vi "Test_Advance_Step_Caraya.vi"(8 "error in":errorcluster) -> (0 "error out":errorcluster)   [LabVIEW 2026]
doc: "Caraya tests of the configurable step phase logic."
uses:
  <vilib>/addons/_JKI Toolkits/Caraya/classes/Test/Test.lvclass
  <vilib>/addons/_JKI Toolkits/Caraya/classes/Assert/Assert.lvclass
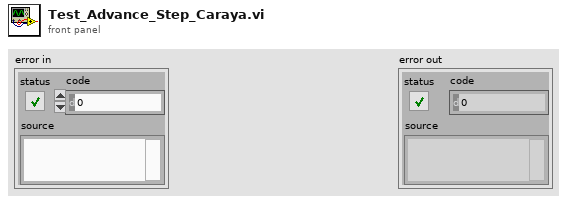
[diagram p1: front panel]
types:
  T1 = cluster{"phase":i32, "phase_start_ms":dbl, "retries":i32}
  T2 = cluster{"step_no":i32, "step_name":string, "interlock_status":string, "pre_delay_ms":dbl, "post_delay_ms":dbl, "timeout_ms":dbl, "popup":cluster{"enabled":bool, "message":string, "type":string, "timeout_ms":dbl}, "retest":cluster{"enabled":bool, "popup":bool, "popup_message":string, "condition":string, "goto_step_no":i32}, "log":cluster{"peak":bool, "average":bool, "event":bool}, "actions":cluster{"do":cluster{"name":string, "on":bool, "mode":string}[], "ao":cluster{"name":string, "value":dbl, "mode":string}[], "misc_write":cluster{"name":string, "on":bool}[], "call":string[]}, "checks":cluster{"di_high":cluster{"and":string[], "or":string[]}, "di_low":cluster{"and":string[], "or":string[]}, "misc_high":cluster{"and":string[], "or":string[]}, "misc_low":cluster{"and":string[], "or":string[]}, "t0_high":cluster{"and":cluster{"name":string, "min":dbl, "max":dbl}[], "or":cluster{"name":string, "min":dbl, "max":dbl}[]}, "t0_low":cluster{"and":cluster{"name":string, "min":dbl, "max":dbl}[], "or":cluster{"name":string, "min":dbl, "max":dbl}[]}, "misc_compare":cluster{"name":string, "compare_with":string, "comparison":string, "tolerance":dbl}[]}}
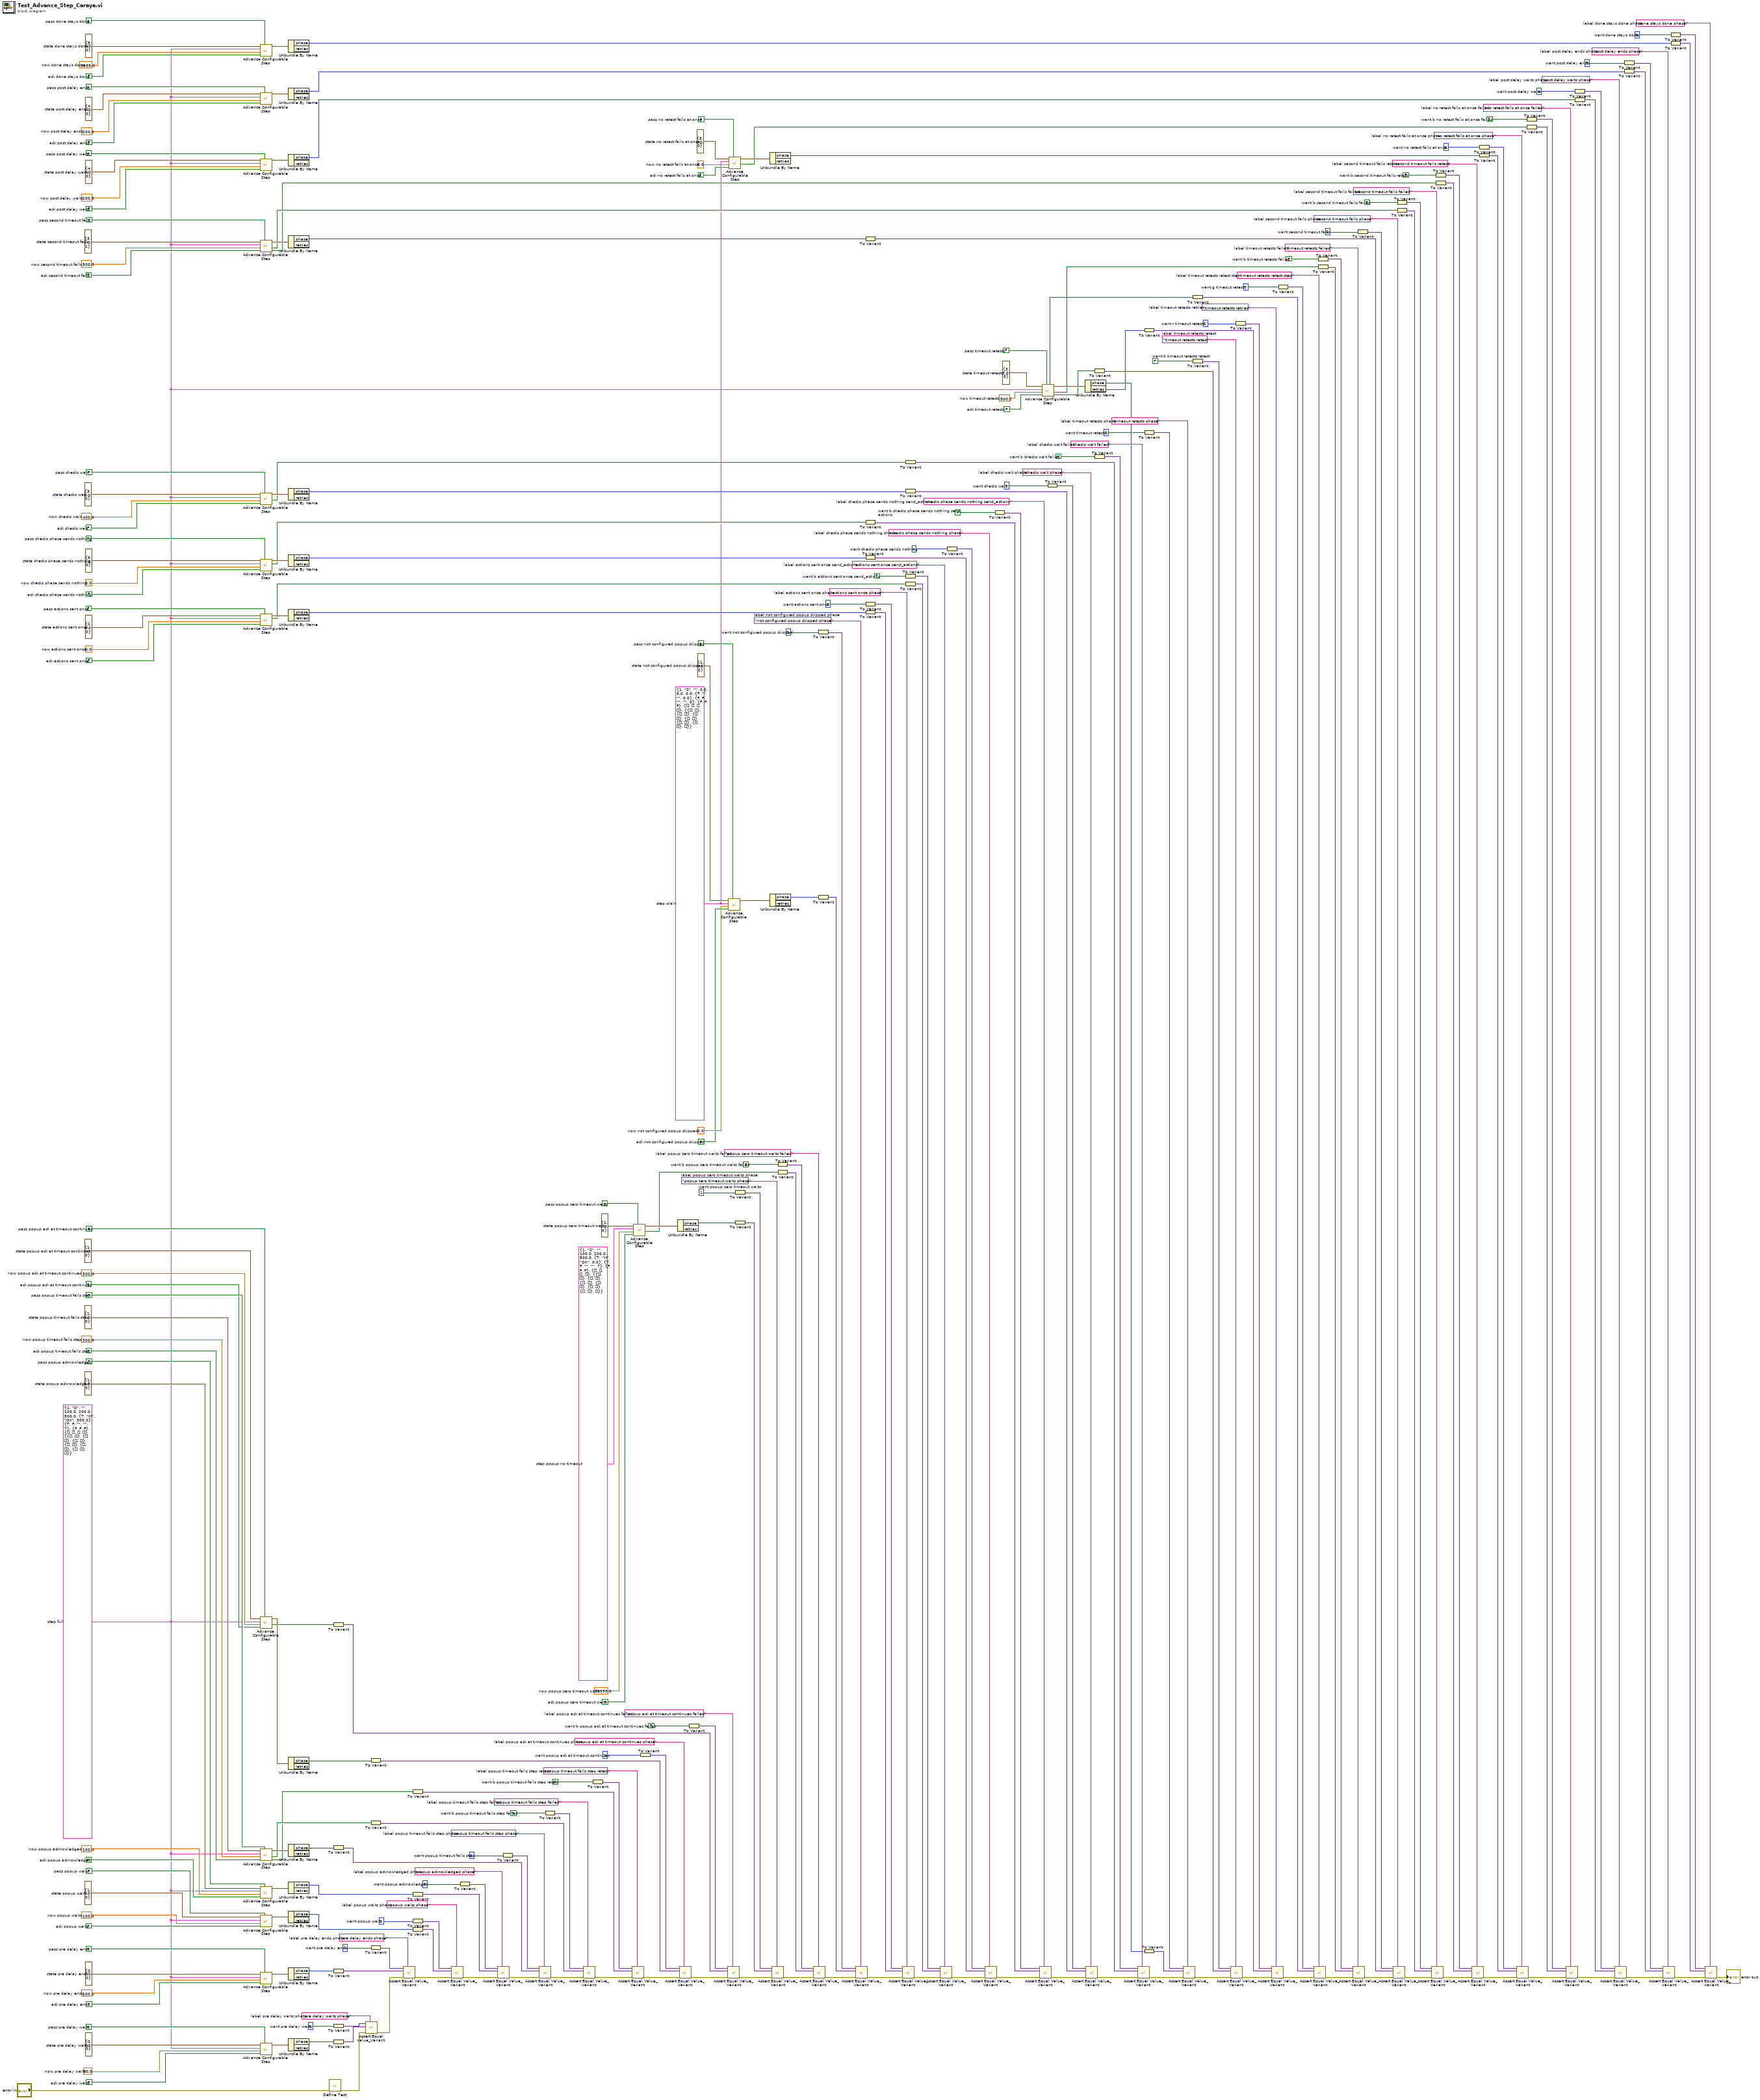
[diagram p0: block diagram]
diagram:
  w5 = "done stays done phase"  # label done stays done phase
  w6 = 5  # want done stays done
  w9 = FALSE  # pass done stays done
  w10 = FALSE  # ack done stays done
  w11 = 9999.0  # now done stays done
  w13 = T1 {"phase"=5, "phase_start_ms"=0.0, "retries"=0}  # state done stays done
  w17 = "post delay ends phase"  # label post delay ends phase
  w18 = 5  # want post delay ends
  w21 = FALSE  # pass post delay ends
  w22 = FALSE  # ack post delay ends
  w23 = 200.0  # now post delay ends
  w24 = T1 {"phase"=4, "phase_start_ms"=0.0, "retries"=0}  # state post delay ends
  w28 = "post delay waits phase"  # label post delay waits phase
  w29 = 4  # want post delay waits
  w32 = FALSE  # pass post delay waits
  w33 = FALSE  # ack post delay waits
  w34 = 100.0  # now post delay waits
  w35 = T1 {"phase"=4, "phase_start_ms"=0.0, "retries"=0}  # state post delay waits
  w39 = "no retest fails at once failed"  # label no retest fails at once failed
  w40 = TRUE  # want b no retest fails at once failed
  w45 = "no retest fails at once phase"  # label no retest fails at once phase
  w46 = 6  # want no retest fails at once
  w49 = FALSE  # pass no retest fails at once
  w50 = FALSE  # ack no retest fails at once
  w51 = 0.0  # now no retest fails at once
  w53 = T1 {"phase"=3, "phase_start_ms"=0.0, "retries"=0}  # state no retest fails at once
  w57 = "second timeout fails retest"  # label second timeout fails retest
  w58 = FALSE  # want b second timeout fails retest
  w63 = "second timeout fails failed"  # label second timeout fails failed
  w64 = TRUE  # want b second timeout fails failed
  w69 = "second timeout fails phase"  # label second timeout fails phase
  w70 = 6  # want second timeout fails
  w73 = FALSE  # pass second timeout fails
  w74 = FALSE  # ack second timeout fails
  w75 = 500.0  # now second timeout fails
  w76 = T1 {"phase"=3, "phase_start_ms"=0.0, "retries"=1}  # state second timeout fails
  w80 = "timeout retests failed"  # label timeout retests failed
  w81 = FALSE  # want b timeout retests failed
  w86 = "timeout retests retest step"  # label timeout retests retest step
  w87 = 7  # want g timeout retests
  w92 = "timeout retests retries"  # label timeout retests retries
  w93 = 1  # want r timeout retests
  w98 = "timeout retests retest"  # label timeout retests retest
  w99 = TRUE  # want b timeout retests retest
  w104 = "timeout retests phase"  # label timeout retests phase
  w105 = 0  # want timeout retests
  w108 = FALSE  # pass timeout retests
  w109 = FALSE  # ack timeout retests
  w110 = 500.0  # now timeout retests
  w111 = T1 {"phase"=3, "phase_start_ms"=0.0, "retries"=0}  # state timeout retests
  w115 = "checks wait failed"  # label checks wait failed
  w116 = FALSE  # want b checks wait failed
  w121 = "checks wait phase"  # label checks wait phase
  w122 = 3  # want checks wait
  w125 = FALSE  # pass checks wait
  w126 = FALSE  # ack checks wait
  w127 = 400.0  # now checks wait
  w128 = T1 {"phase"=3, "phase_start_ms"=0.0, "retries"=0}  # state checks wait
  w132 = "checks phase sends nothing send_actions"  # label checks phase sends nothing send_actions
  w133 = FALSE  # want b checks phase sends nothing send_actions
  w138 = "checks phase sends nothing phase"  # label checks phase sends nothing phase
  w139 = 4  # want checks phase sends nothing
  w142 = TRUE  # pass checks phase sends nothing
  w143 = FALSE  # ack checks phase sends nothing
  w144 = 0.0  # now checks phase sends nothing
  w145 = T1 {"phase"=3, "phase_start_ms"=0.0, "retries"=0}  # state checks phase sends nothing
  w149 = "actions sent once send_actions"  # label actions sent once send_actions
  w150 = TRUE  # want b actions sent once send_actions
  w155 = "actions sent once phase"  # label actions sent once phase
  w156 = 3  # want actions sent once
  w159 = FALSE  # pass actions sent once
  w160 = FALSE  # ack actions sent once
  w161 = 0.0  # now actions sent once
  w162 = T1 {"phase"=2, "phase_start_ms"=0.0, "retries"=0}  # state actions sent once
  w166 = "not configured popup skipped phase"  # label not configured popup skipped phase
  w167 = 2  # want not configured popup skipped
  w170 = FALSE  # pass not configured popup skipped
  w171 = FALSE  # ack not configured popup skipped
  w172 = 0.0  # now not configured popup skipped
  w173 = T1 {"phase"=1, "phase_start_ms"=0.0, "retries"=0}  # state not configured popup skipped
  w177 = "popup zero timeout waits failed"  # label popup zero timeout waits failed
  w178 = FALSE  # want b popup zero timeout waits failed
  w183 = "popup zero timeout waits phase"  # label popup zero timeout waits phase
  w184 = 1  # want popup zero timeout waits
  w187 = FALSE  # pass popup zero timeout waits
  w188 = FALSE  # ack popup zero timeout waits
  w189 = 99999.0  # now popup zero timeout waits
  w191 = T1 {"phase"=1, "phase_start_ms"=0.0, "retries"=0}  # state popup zero timeout waits
  w190 = T2 {"step_no"=1, "step_name"="S", "interlock_status"="", "pre_delay_ms"=100.0, "post_delay_ms"=200.0, "timeout_ms"=500.0, "popup"={"enabled"=TRUE, "message"="M", "type"="OK", "timeout_ms"=0.0}, "retest"={"enabled"=TRUE, "popup"=FALSE, "popup_message"="", "condition"="", "goto_step_no"=7}, "log"={"peak"=FALSE, "average"=FALSE, "event"=FALSE}, "actions"={"do"=[], "ao"=[], "misc_write"=[], "call"=[]}, "checks"={"di_high"={"and"=[], "or"=[]}, "di_low"={"and"=[], "or"=[]}, "misc_high"={"and"=[], "or"=[]}, "misc_low"={"and"=[], "or"=[]}, "t0_high"={"and"=[], "or"=[]}, "t0_low"={"and"=[], "or"=[]}, "misc_compare"=[]}}  # step popup no timeout
  w195 = "popup ack at timeout continues failed"  # label popup ack at timeout continues failed
  w196 = FALSE  # want b popup ack at timeout continues failed
  w201 = "popup ack at timeout continues phase"  # label popup ack at timeout continues phase
  w202 = 2  # want popup ack at timeout continues
  w205 = FALSE  # pass popup ack at timeout continues
  w206 = TRUE  # ack popup ack at timeout continues
  w207 = 300.0  # now popup ack at timeout continues
  w208 = T1 {"phase"=1, "phase_start_ms"=0.0, "retries"=0}  # state popup ack at timeout continues
  w212 = "popup timeout fails step retest"  # label popup timeout fails step retest
  w213 = FALSE  # want b popup timeout fails step retest
  w218 = "popup timeout fails step failed"  # label popup timeout fails step failed
  w219 = TRUE  # want b popup timeout fails step failed
  w224 = "popup timeout fails step phase"  # label popup timeout fails step phase
  w225 = 6  # want popup timeout fails step
  w228 = FALSE  # pass popup timeout fails step
  w229 = FALSE  # ack popup timeout fails step
  w230 = 300.0  # now popup timeout fails step
  w231 = T1 {"phase"=1, "phase_start_ms"=0.0, "retries"=0}  # state popup timeout fails step
  w235 = "popup acknowledged phase"  # label popup acknowledged phase
  w236 = 2  # want popup acknowledged
  w239 = FALSE  # pass popup acknowledged
  w240 = TRUE  # ack popup acknowledged
  w241 = 100.0  # now popup acknowledged
  w242 = T1 {"phase"=1, "phase_start_ms"=0.0, "retries"=0}  # state popup acknowledged
  w246 = "popup waits phase"  # label popup waits phase
  w247 = 1  # want popup waits
  w250 = FALSE  # pass popup waits
  w251 = FALSE  # ack popup waits
  w252 = 100.0  # now popup waits
  w253 = T1 {"phase"=1, "phase_start_ms"=0.0, "retries"=0}  # state popup waits
  w257 = "pre delay ends phase"  # label pre delay ends phase
  w258 = 1  # want pre delay ends
  w261 = FALSE  # pass pre delay ends
  w262 = FALSE  # ack pre delay ends
  w263 = 100.0  # now pre delay ends
  w264 = T1 {"phase"=0, "phase_start_ms"=0.0, "retries"=0}  # state pre delay ends
  w268 = "pre delay waits phase"  # label pre delay waits phase
  w269 = 0  # want pre delay waits
  w272 = FALSE  # pass pre delay waits
  w273 = FALSE  # ack pre delay waits
  w274 = 50.0  # now pre delay waits
  w275 = T1 {"phase"=0, "phase_start_ms"=0.0, "retries"=0}  # state pre delay waits
  w52 = T2 {"step_no"=1, "step_name"="S", "interlock_status"="", "pre_delay_ms"=0.0, "post_delay_ms"=0.0, "timeout_ms"=0.0, "popup"={"enabled"=FALSE, "message"="", "type"="", "timeout_ms"=0.0}, "retest"={"enabled"=FALSE, "popup"=FALSE, "popup_message"="", "condition"="", "goto_step_no"=0}, "log"={"peak"=FALSE, "average"=FALSE, "event"=FALSE}, "actions"={"do"=[], "ao"=[], "misc_write"=[], "call"=[]}, "checks"={"di_high"={"and"=[], "or"=[]}, "di_low"={"and"=[], "or"=[]}, "misc_high"={"and"=[], "or"=[]}, "misc_low"={"and"=[], "or"=[]}, "t0_high"={"and"=[], "or"=[]}, "t0_low"={"and"=[], "or"=[]}, "misc_compare"=[]}}  # step plain
  w12 = T2 {"step_no"=1, "step_name"="S", "interlock_status"="", "pre_delay_ms"=100.0, "post_delay_ms"=200.0, "timeout_ms"=500.0, "popup"={"enabled"=TRUE, "message"="M", "type"="OK", "timeout_ms"=300.0}, "retest"={"enabled"=TRUE, "popup"=FALSE, "popup_message"="", "condition"="", "goto_step_no"=7}, "log"={"peak"=FALSE, "average"=FALSE, "event"=FALSE}, "actions"={"do"=[], "ao"=[], "misc_write"=[], "call"=[]}, "checks"={"di_high"={"and"=[], "or"=[]}, "di_low"={"and"=[], "or"=[]}, "misc_high"={"and"=[], "or"=[]}, "misc_low"={"and"=[], "or"=[]}, "t0_high"={"and"=[], "or"=[]}, "t0_low"={"and"=[], "or"=[]}, "misc_compare"=[]}}  # step full
  n1 = call "Advance Configurable Step.vi"("checks passed"=w9, "popup acknowledged"=w10, "now ms"=w11, "Step"=w12, "State"=w13) -> ("Next State"=w8:T1)  [unwired: 2 in, 4 out]
  n2 = call "Advance Configurable Step.vi"("checks passed"=w21, "popup acknowledged"=w22, "now ms"=w23, "Step"=w12, "State"=w24) -> ("Next State"=w20:T1)  [unwired: 2 in, 4 out]
  n3 = call "Advance Configurable Step.vi"("checks passed"=w32, "popup acknowledged"=w33, "now ms"=w34, "Step"=w12, "State"=w35) -> ("Next State"=w31:T1)  [unwired: 2 in, 4 out]
  n4 = call "Advance Configurable Step.vi"("checks passed"=w73, "popup acknowledged"=w74, "now ms"=w75, "Step"=w12, "State"=w76) -> ("retest"=w59:bool, "failed"=w65:bool, "Next State"=w72:T1)  [unwired: 2 in, 2 out]
  n5 = call "Advance Configurable Step.vi"("checks passed"=w125, "popup acknowledged"=w126, "now ms"=w127, "Step"=w12, "State"=w128) -> ("failed"=w117:bool, "Next State"=w124:T1)  [unwired: 2 in, 3 out]
  n6 = call "Advance Configurable Step.vi"("checks passed"=w142, "popup acknowledged"=w143, "now ms"=w144, "Step"=w12, "State"=w145) -> ("send actions"=w134:bool, "Next State"=w141:T1)  [unwired: 2 in, 3 out]
  n7 = call "Advance Configurable Step.vi"("checks passed"=w159, "popup acknowledged"=w160, "now ms"=w161, "Step"=w12, "State"=w162) -> ("send actions"=w151:bool, "Next State"=w158:T1)  [unwired: 2 in, 3 out]
  n8 = call "Advance Configurable Step.vi"("checks passed"=w205, "popup acknowledged"=w206, "now ms"=w207, "Step"=w12, "State"=w208) -> ("failed"=w197:bool, "Next State"=w204:T1)  [unwired: 2 in, 3 out]
  n9 = call "Advance Configurable Step.vi"("checks passed"=w228, "popup acknowledged"=w229, "now ms"=w230, "Step"=w12, "State"=w231) -> ("retest"=w214:bool, "failed"=w220:bool, "Next State"=w227:T1)  [unwired: 2 in, 2 out]
  n10 = call "Advance Configurable Step.vi"("checks passed"=w239, "popup acknowledged"=w240, "now ms"=w241, "Step"=w12, "State"=w242) -> ("Next State"=w238:T1)  [unwired: 2 in, 4 out]
  n11 = call "Advance Configurable Step.vi"("checks passed"=w250, "popup acknowledged"=w251, "now ms"=w252, "Step"=w12, "State"=w253) -> ("Next State"=w249:T1)  [unwired: 2 in, 4 out]
  n12 = call "Advance Configurable Step.vi"("checks passed"=w261, "popup acknowledged"=w262, "now ms"=w263, "Step"=w12, "State"=w264) -> ("Next State"=w260:T1)  [unwired: 2 in, 4 out]
  n13 = call "Advance Configurable Step.vi"("checks passed"=w272, "popup acknowledged"=w273, "now ms"=w274, "Step"=w12, "State"=w275) -> ("Next State"=w271:T1)  [unwired: 2 in, 4 out]
  n14 = Unbundle By Name(w8) -> ("phase"=w7:i32)  [unwired: 1 out]
  n15 = Unbundle By Name(w20) -> ("phase"=w19:i32)  [unwired: 1 out]
  n16 = Unbundle By Name(w31) -> ("phase"=w30:i32)  [unwired: 1 out]
  n17 = Unbundle By Name(w72) -> ("phase"=w71:i32)  [unwired: 1 out]
  n18 = Unbundle By Name(w124) -> ("phase"=w123:i32)  [unwired: 1 out]
  n19 = Unbundle By Name(w141) -> ("phase"=w140:i32)  [unwired: 1 out]
  n20 = Unbundle By Name(w158) -> ("phase"=w157:i32)  [unwired: 1 out]
  n21 = Unbundle By Name(w204) -> ("phase"=w203:i32)  [unwired: 1 out]
  n22 = Unbundle By Name(w227) -> ("phase"=w226:i32)  [unwired: 1 out]
  n23 = Unbundle By Name(w238) -> ("phase"=w237:i32)  [unwired: 1 out]
  n24 = Unbundle By Name(w249) -> ("phase"=w248:i32)  [unwired: 1 out]
  n25 = Unbundle By Name(w260) -> ("phase"=w259:i32)  [unwired: 1 out]
  n26 = Unbundle By Name(w271) -> ("phase"=w270:i32)  [unwired: 1 out]
  n27 = call <vilib>:"Define Test.vi"("error in (no error)"="error in") -> ("error out"=w267:errorcluster)  [unwired: 9 in, 1 out]
  n28 = To Variant(anything=w197) -> (Variant=w193:variant)
  n29 = To Variant(anything=w226) -> (Variant=w222:variant)
  n30 = To Variant(anything=w259) -> (Variant=w255:variant)
  n31 = To Variant(anything=w269) -> (Variant=w265:variant)
  n32 = To Variant(anything=w270) -> (Variant=w266:variant)
  n33 = call <vilib>:"Assert Equal Value_Variant.vi"("Label"=w268, "error in (no error)"=w267, "Actual"=w266, "Expected"=w265) -> ("error out"=w256:errorcluster)  [unwired: 6 in, 1 out]
  n34 = To Variant(anything=w203) -> (Variant=w199:variant)
  n35 = To Variant(anything=w220) -> (Variant=w216:variant)
  n36 = To Variant(anything=w258) -> (Variant=w254:variant)
  n37 = call <vilib>:"Assert Equal Value_Variant.vi"("Label"=w257, "error in (no error)"=w256, "Actual"=w255, "Expected"=w254) -> ("error out"=w245:errorcluster)  [unwired: 6 in, 1 out]
  n38 = To Variant(anything=w214) -> (Variant=w210:variant)
  n39 = To Variant(anything=w237) -> (Variant=w233:variant)
  n40 = To Variant(anything=w247) -> (Variant=w243:variant)
  n41 = To Variant(anything=w248) -> (Variant=w244:variant)
  n42 = call <vilib>:"Assert Equal Value_Variant.vi"("Label"=w246, "error in (no error)"=w245, "Actual"=w244, "Expected"=w243) -> ("error out"=w234:errorcluster)  [unwired: 6 in, 1 out]
  n43 = To Variant(anything=w236) -> (Variant=w232:variant)
  n44 = call <vilib>:"Assert Equal Value_Variant.vi"("Label"=w235, "error in (no error)"=w234, "Actual"=w233, "Expected"=w232) -> ("error out"=w223:errorcluster)  [unwired: 6 in, 1 out]
  n45 = To Variant(anything=w225) -> (Variant=w221:variant)
  n46 = call <vilib>:"Assert Equal Value_Variant.vi"("Label"=w224, "error in (no error)"=w223, "Actual"=w222, "Expected"=w221) -> ("error out"=w217:errorcluster)  [unwired: 6 in, 1 out]
  n47 = To Variant(anything=w219) -> (Variant=w215:variant)
  n48 = call <vilib>:"Assert Equal Value_Variant.vi"("Label"=w218, "error in (no error)"=w217, "Actual"=w216, "Expected"=w215) -> ("error out"=w211:errorcluster)  [unwired: 6 in, 1 out]
  n49 = To Variant(anything=w213) -> (Variant=w209:variant)
  n50 = call <vilib>:"Assert Equal Value_Variant.vi"("Label"=w212, "error in (no error)"=w211, "Actual"=w210, "Expected"=w209) -> ("error out"=w200:errorcluster)  [unwired: 6 in, 1 out]
  n51 = call "Advance Configurable Step.vi"("checks passed"=w187, "popup acknowledged"=w188, "now ms"=w189, "Step"=w190, "State"=w191) -> ("failed"=w179:bool, "Next State"=w186:T1)  [unwired: 2 in, 3 out]
  n52 = To Variant(anything=w202) -> (Variant=w198:variant)
  n53 = Unbundle By Name(w186) -> ("phase"=w185:i32)  [unwired: 1 out]
  n54 = call <vilib>:"Assert Equal Value_Variant.vi"("Label"=w201, "error in (no error)"=w200, "Actual"=w199, "Expected"=w198) -> ("error out"=w194:errorcluster)  [unwired: 6 in, 1 out]
  n55 = To Variant(anything=w196) -> (Variant=w192:variant)
  n56 = call <vilib>:"Assert Equal Value_Variant.vi"("Label"=w195, "error in (no error)"=w194, "Actual"=w193, "Expected"=w192) -> ("error out"=w182:errorcluster)  [unwired: 6 in, 1 out]
  n57 = call "Advance Configurable Step.vi"("checks passed"=w170, "popup acknowledged"=w171, "now ms"=w172, "Step"=w52, "State"=w173) -> ("Next State"=w169:T1)  [unwired: 2 in, 4 out]
  n58 = call "Advance Configurable Step.vi"("checks passed"=w49, "popup acknowledged"=w50, "now ms"=w51, "Step"=w52, "State"=w53) -> ("failed"=w41:bool, "Next State"=w48:T1)  [unwired: 2 in, 3 out]
  n59 = To Variant(anything=w184) -> (Variant=w180:variant)
  n60 = To Variant(anything=w185) -> (Variant=w181:variant)
  n61 = Unbundle By Name(w48) -> ("phase"=w47:i32)  [unwired: 1 out]
  n62 = Unbundle By Name(w169) -> ("phase"=w168:i32)  [unwired: 1 out]
  n63 = call <vilib>:"Assert Equal Value_Variant.vi"("Label"=w183, "error in (no error)"=w182, "Actual"=w181, "Expected"=w180) -> ("error out"=w176:errorcluster)  [unwired: 6 in, 1 out]
  n64 = To Variant(anything=w178) -> (Variant=w174:variant)
  n65 = To Variant(anything=w179) -> (Variant=w175:variant)
  n66 = call <vilib>:"Assert Equal Value_Variant.vi"("Label"=w177, "error in (no error)"=w176, "Actual"=w175, "Expected"=w174) -> ("error out"=w165:errorcluster)  [unwired: 6 in, 1 out]
  n67 = To Variant(anything=w167) -> (Variant=w163:variant)
  n68 = To Variant(anything=w168) -> (Variant=w164:variant)
  n69 = call <vilib>:"Assert Equal Value_Variant.vi"("Label"=w166, "error in (no error)"=w165, "Actual"=w164, "Expected"=w163) -> ("error out"=w154:errorcluster)  [unwired: 6 in, 1 out]
  n70 = To Variant(anything=w71) -> (Variant=w67:variant)
  n71 = To Variant(anything=w134) -> (Variant=w130:variant)
  n72 = To Variant(anything=w140) -> (Variant=w136:variant)
  n73 = To Variant(anything=w156) -> (Variant=w152:variant)
  n74 = To Variant(anything=w157) -> (Variant=w153:variant)
  n75 = call <vilib>:"Assert Equal Value_Variant.vi"("Label"=w155, "error in (no error)"=w154, "Actual"=w153, "Expected"=w152) -> ("error out"=w148:errorcluster)  [unwired: 6 in, 1 out]
  n76 = To Variant(anything=w117) -> (Variant=w113:variant)
  n77 = To Variant(anything=w123) -> (Variant=w119:variant)
  n78 = To Variant(anything=w150) -> (Variant=w146:variant)
  n79 = To Variant(anything=w151) -> (Variant=w147:variant)
  n80 = call <vilib>:"Assert Equal Value_Variant.vi"("Label"=w149, "error in (no error)"=w148, "Actual"=w147, "Expected"=w146) -> ("error out"=w137:errorcluster)  [unwired: 6 in, 1 out]
  n81 = To Variant(anything=w139) -> (Variant=w135:variant)
  n82 = call <vilib>:"Assert Equal Value_Variant.vi"("Label"=w138, "error in (no error)"=w137, "Actual"=w136, "Expected"=w135) -> ("error out"=w131:errorcluster)  [unwired: 6 in, 1 out]
  n83 = To Variant(anything=w133) -> (Variant=w129:variant)
  n84 = call <vilib>:"Assert Equal Value_Variant.vi"("Label"=w132, "error in (no error)"=w131, "Actual"=w130, "Expected"=w129) -> ("error out"=w120:errorcluster)  [unwired: 6 in, 1 out]
  n85 = call "Advance Configurable Step.vi"("checks passed"=w108, "popup acknowledged"=w109, "now ms"=w110, "Step"=w12, "State"=w111) -> ("retest"=w100:bool, "failed"=w82:bool, "Next State"=w107:T1, "retest step"=w88:i32)  [unwired: 2 in, 1 out]
  n86 = To Variant(anything=w122) -> (Variant=w118:variant)
  n87 = Unbundle By Name(w107) -> ("phase"=w106:i32, "retries"=w94:i32)
  n88 = call <vilib>:"Assert Equal Value_Variant.vi"("Label"=w121, "error in (no error)"=w120, "Actual"=w119, "Expected"=w118) -> ("error out"=w114:errorcluster)  [unwired: 6 in, 1 out]
  n89 = To Variant(anything=w100) -> (Variant=w96:variant)
  n90 = To Variant(anything=w116) -> (Variant=w112:variant)
  n91 = call <vilib>:"Assert Equal Value_Variant.vi"("Label"=w115, "error in (no error)"=w114, "Actual"=w113, "Expected"=w112) -> ("error out"=w103:errorcluster)  [unwired: 6 in, 1 out]
  n92 = To Variant(anything=w94) -> (Variant=w90:variant)
  n93 = To Variant(anything=w105) -> (Variant=w101:variant)
  n94 = To Variant(anything=w106) -> (Variant=w102:variant)
  n95 = call <vilib>:"Assert Equal Value_Variant.vi"("Label"=w104, "error in (no error)"=w103, "Actual"=w102, "Expected"=w101) -> ("error out"=w97:errorcluster)  [unwired: 6 in, 1 out]
  n96 = To Variant(anything=w88) -> (Variant=w84:variant)
  n97 = To Variant(anything=w99) -> (Variant=w95:variant)
  n98 = call <vilib>:"Assert Equal Value_Variant.vi"("Label"=w98, "error in (no error)"=w97, "Actual"=w96, "Expected"=w95) -> ("error out"=w91:errorcluster)  [unwired: 6 in, 1 out]
  n99 = To Variant(anything=w93) -> (Variant=w89:variant)
  n100 = call <vilib>:"Assert Equal Value_Variant.vi"("Label"=w92, "error in (no error)"=w91, "Actual"=w90, "Expected"=w89) -> ("error out"=w85:errorcluster)  [unwired: 6 in, 1 out]
  n101 = To Variant(anything=w87) -> (Variant=w83:variant)
  n102 = call <vilib>:"Assert Equal Value_Variant.vi"("Label"=w86, "error in (no error)"=w85, "Actual"=w84, "Expected"=w83) -> ("error out"=w79:errorcluster)  [unwired: 6 in, 1 out]
  n103 = To Variant(anything=w81) -> (Variant=w77:variant)
  n104 = To Variant(anything=w82) -> (Variant=w78:variant)
  n105 = call <vilib>:"Assert Equal Value_Variant.vi"("Label"=w80, "error in (no error)"=w79, "Actual"=w78, "Expected"=w77) -> ("error out"=w68:errorcluster)  [unwired: 6 in, 1 out]
  n106 = To Variant(anything=w70) -> (Variant=w66:variant)
  n107 = call <vilib>:"Assert Equal Value_Variant.vi"("Label"=w69, "error in (no error)"=w68, "Actual"=w67, "Expected"=w66) -> ("error out"=w62:errorcluster)  [unwired: 6 in, 1 out]
  n108 = To Variant(anything=w64) -> (Variant=w60:variant)
  n109 = To Variant(anything=w65) -> (Variant=w61:variant)
  n110 = call <vilib>:"Assert Equal Value_Variant.vi"("Label"=w63, "error in (no error)"=w62, "Actual"=w61, "Expected"=w60) -> ("error out"=w56:errorcluster)  [unwired: 6 in, 1 out]
  n111 = To Variant(anything=w58) -> (Variant=w54:variant)
  n112 = To Variant(anything=w59) -> (Variant=w55:variant)
  n113 = call <vilib>:"Assert Equal Value_Variant.vi"("Label"=w57, "error in (no error)"=w56, "Actual"=w55, "Expected"=w54) -> ("error out"=w44:errorcluster)  [unwired: 6 in, 1 out]
  n114 = To Variant(anything=w46) -> (Variant=w42:variant)
  n115 = To Variant(anything=w47) -> (Variant=w43:variant)
  n116 = call <vilib>:"Assert Equal Value_Variant.vi"("Label"=w45, "error in (no error)"=w44, "Actual"=w43, "Expected"=w42) -> ("error out"=w38:errorcluster)  [unwired: 6 in, 1 out]
  n117 = To Variant(anything=w40) -> (Variant=w36:variant)
  n118 = To Variant(anything=w41) -> (Variant=w37:variant)
  n119 = call <vilib>:"Assert Equal Value_Variant.vi"("Label"=w39, "error in (no error)"=w38, "Actual"=w37, "Expected"=w36) -> ("error out"=w27:errorcluster)  [unwired: 6 in, 1 out]
  n120 = To Variant(anything=w29) -> (Variant=w25:variant)
  n121 = To Variant(anything=w30) -> (Variant=w26:variant)
  n122 = call <vilib>:"Assert Equal Value_Variant.vi"("Label"=w28, "error in (no error)"=w27, "Actual"=w26, "Expected"=w25) -> ("error out"=w16:errorcluster)  [unwired: 6 in, 1 out]
  n123 = To Variant(anything=w18) -> (Variant=w14:variant)
  n124 = To Variant(anything=w19) -> (Variant=w15:variant)
  n125 = call <vilib>:"Assert Equal Value_Variant.vi"("Label"=w17, "error in (no error)"=w16, "Actual"=w15, "Expected"=w14) -> ("error out"=w4:errorcluster)  [unwired: 6 in, 1 out]
  n126 = To Variant(anything=w6) -> (Variant=w2:variant)
  n127 = To Variant(anything=w7) -> (Variant=w3:variant)
  n128 = call <vilib>:"Assert Equal Value_Variant.vi"("Label"=w5, "error in (no error)"=w4, "Actual"=w3, "Expected"=w2) -> ("error out"=→"error out":errorcluster)  [unwired: 6 in, 1 out]
